vi "gen pulse.vi"(6 "clk per pulse":u32, 7 "bit":u8=1, 8 "Motor Pulse Rate / mm":i32, 9 "kx":dbl=1.0, 10 "xn":dbl=1000.0, 11 "dir":bool) -> (1 "pulsetrain":u8[](graph), 2 "s curve":u32[](graph), 3 "raw s curve":u32[](graph))   [LabVIEW 2024]
panel:
  out "Numeric 2":dbl
  in  "en":bool=TRUE
  out "Numeric":i32
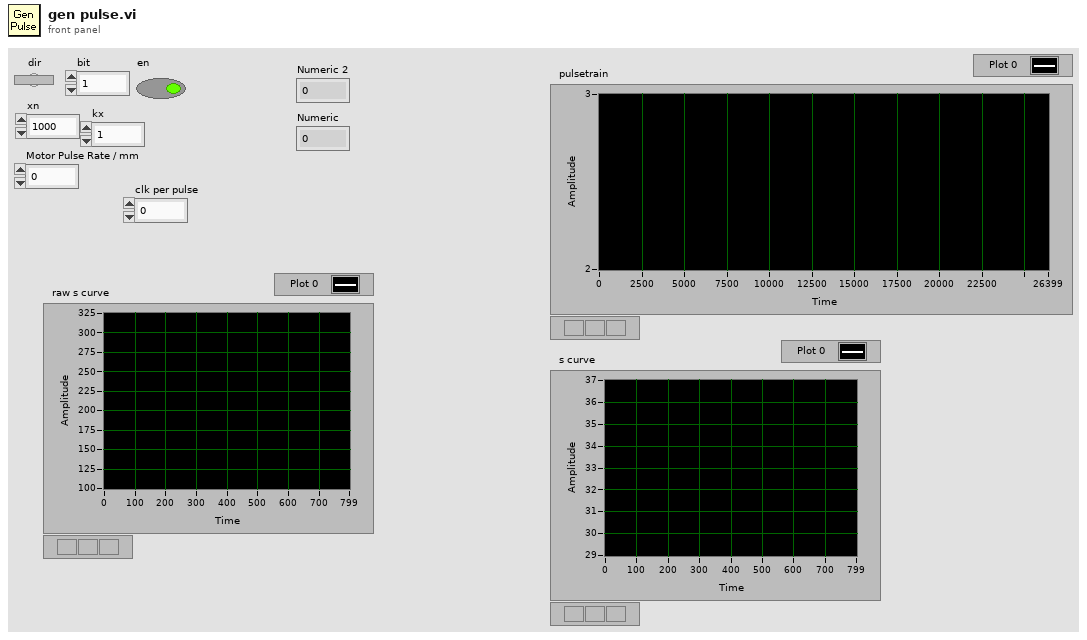
[diagram p1: front panel]
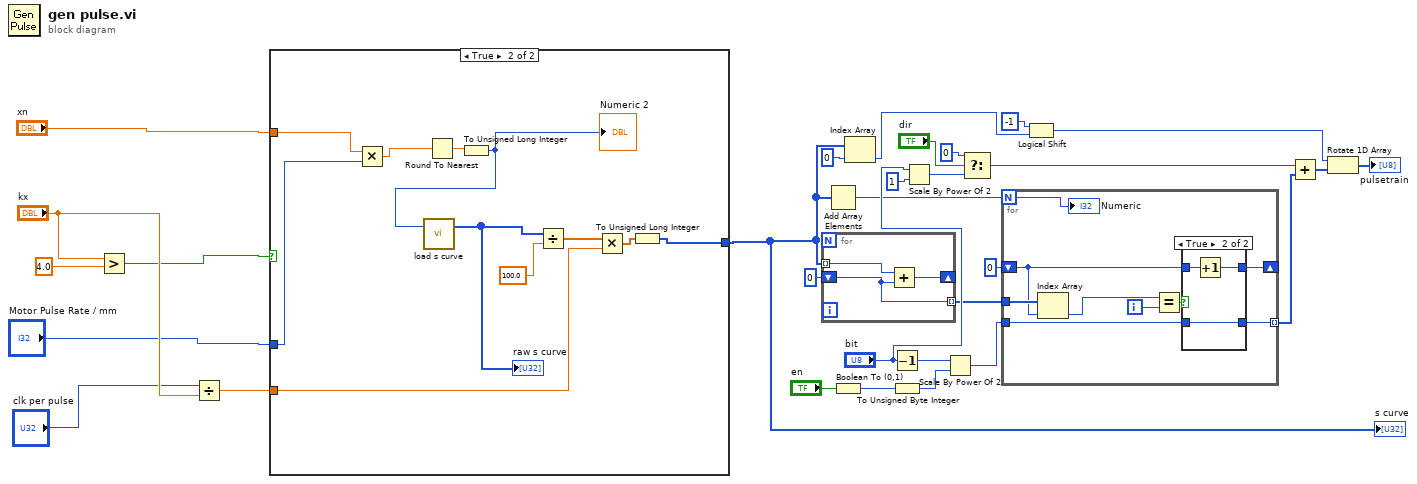
[diagram p0: block diagram]
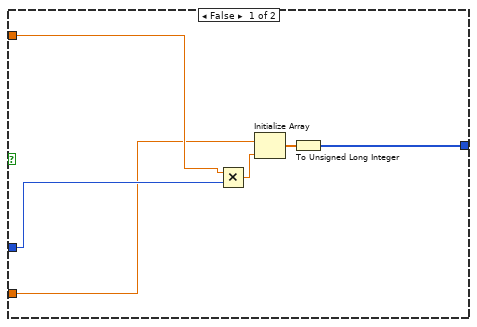
[diagram p2: hidden frame]
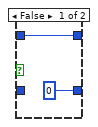
[diagram p3: hidden frame]
diagram:
  n1 = Greater?(x="kx", y=4.0) -> (0:w6:bool)
  n2 = Divide(x="clk per pulse", y="kx") -> (x/y=w2:dbl)
  n3 = case shown="True" w6 {
    tunnel: "xn" -> [w36 w47]
    tunnel: [w33 w43] -> w4
    tunnel: "Motor Pulse Rate / mm" -> [w32 w44]
    tunnel: w2 -> [w31 w37]
    frame False {
      n4 = Multiply(x=w36, y=w32) -> (x*y=w35:dbl)
      n5 = Initialize Array(w31, w35) -> (w34:dbl[])
      n6 = To Unsigned Long Integer(number=w34) -> (unsigned 32bit integer=w33:u32[])
    }
    frame True {
      n7 = Multiply(x=w47, y=w44) -> (x*y=w46:dbl)
      n8 = Round To Nearest(number=w46) -> (nearest integer value=w45:dbl)
      n9 = To Unsigned Long Integer(number=w45) -> (unsigned 32bit integer=w42:u32)
      "Numeric 2" <- w42
      n10 = call "load s curve.vi"("pulses"=w42) -> ("Raw S Curve"=w41:u32[])  [unwired: 2 in]
      "raw s curve" <- w41
      n11 = Divide(x=w41, y=100.0) -> (x/y=w38:dbl[])
      n12 = Multiply(x=w38, y=w37) -> (x*y=w39:dbl[])
      n13 = To Unsigned Long Integer(number=w39) -> (unsigned 32bit integer=w43:u32[])
    }
  }
  "s curve" <- w4
  n14 = for {
    tunnel: w4 -> [w50] mode=indexing
    shift-right: [w49] -> _
    shift-left: u32 0 -> [w48]
    tunnel: [w48] -> w11 mode=indexing
    n15 = Add(x=w50, y=w48) -> (x+y=w49:u32)
  }
  n16 = Add Array Elements(numeric array=w4) -> (sum=w3:u32)
  n17 = Boolean To (0,1)(Boolean="en") -> (0, 1=w18:i16)
  n18 = Index Array(array=w4, index=0) -> (element=w15:u32)
  n19 = Decrement(x="bit") -> (x-1=w27:u8)
  n20 = To Unsigned Byte Integer(number=w18) -> (unsigned 8bit integer=w17:u8)
  n21 = Scale By Power Of 2(n="bit", x=u8 1) -> (x*2^n=w23:u8)
  n22 = Scale By Power Of 2(n=w27, x=w17) -> (x*2^n=w26:u8)
  n23 = Select(t=u8 0 ("element"), s="dir", f=w23) -> (s? t:f=w29:u8)
  n24 = for {
    N: w3 -> [w53]
    tunnel: w11 -> [w59]
    tunnel: w26 -> [w57]
    shift-right: [w54] -> _
    shift-left: u32 0 ("element") -> [w56]
    tunnel: [w55] -> w21 mode=indexing
    i -> [w52]
    n25 = Index Array(array=w59, index=w56) -> (element=w51:u32)
    n26 = Equal?(x=w51, y=w52) -> (x = y?=w58:bool)
    n27 = case shown="True" w58 {
      tunnel: w57 -> [_ w63]
      tunnel: [u8 0 ("element") w63] -> w55
      tunnel: w56 -> [w60 w64]
      tunnel: [w60 w62] -> w54
      frame False {
      }
      frame True {
        n28 = Increment(x=w64) -> (x+1=w62:u32)
      }
    }
    "Numeric" <- w53
  }
  n29 = Logical Shift(y=i16 -1, x=w15) -> (x << y=w13:u32)
  n30 = Add(x=w29, y=w21) -> (x+y=w12:u8[])
  n31 = Rotate 1D Array(1:w12, 2:w13) -> (0:→"pulsetrain":u8[])
